vi "Galvo-Control-V3.vi"() -> ()   [LabVIEW 2024]
uses:
  <vilib>/DAQmx/write.llb/DAQmx Write (Analog 2D DBL NChan NSamp).vi
  <vilib>/DAQmx/write.llb/DAQmx Write (Analog 1D DBL NChan 1Samp).vi
  <vilib>/DAQmx/create/channels.llb/DAQmx Create Channel (AO-Voltage-Basic).vi
  <vilib>/DAQmx/miscellaneous.llb/DAQmx Fill In Error Info.vi
  <vilib>/measure/NI_MABase.lvlib
panel:
  out "element":dbl
  out "size(s)":i32
  out "Random Data (Feedback Node) 3":dbl[](graph)
  out "Random Data (Feedback Node) 2":dbl[](graph)
  out "Random Data (Feedback Node)":dbl[](graph)
  out "Y MIN":dbl
  out "Y MAX":dbl
  out "X MIN":dbl
  out "X MAX":dbl
  out "Waveform Chart":waveform(dbl)(graph)
  out "Waveform Chart 2":waveform(dbl)(graph)
  in  "offset X":dbl format="%0.2p"
  in  "amplitude X":dbl=1.0 format="%0.2p"
  in  "phase":dbl format="%.2p"
  in  "amplitude Y":dbl=1.0 format="%0.2p"
  in  "phase 2":dbl format="%.2p"
  in  "offset Y":dbl format="%0.2p"
  in  "COMMENCE SCAN":bool
  in  "Y desired voltage step(V/100)":dbl=1.0 format="%#_13g"
  in  "X desired voltage step(V/100)":dbl=1.0 format="%#_13g"
  out "Virtual Y position":dbl(graph)
  out "virtual X position":dbl(graph)
  out "Y position":dbl
  out "X position.":dbl
  # "This VI is intended for the user to first define a\nrectangular region to scan, and then to commence\nthe scan at some desired resolution.\n\nthe resolution is defined using the voltage step controls\n\nthe amplitude and offset controls define the scan region"
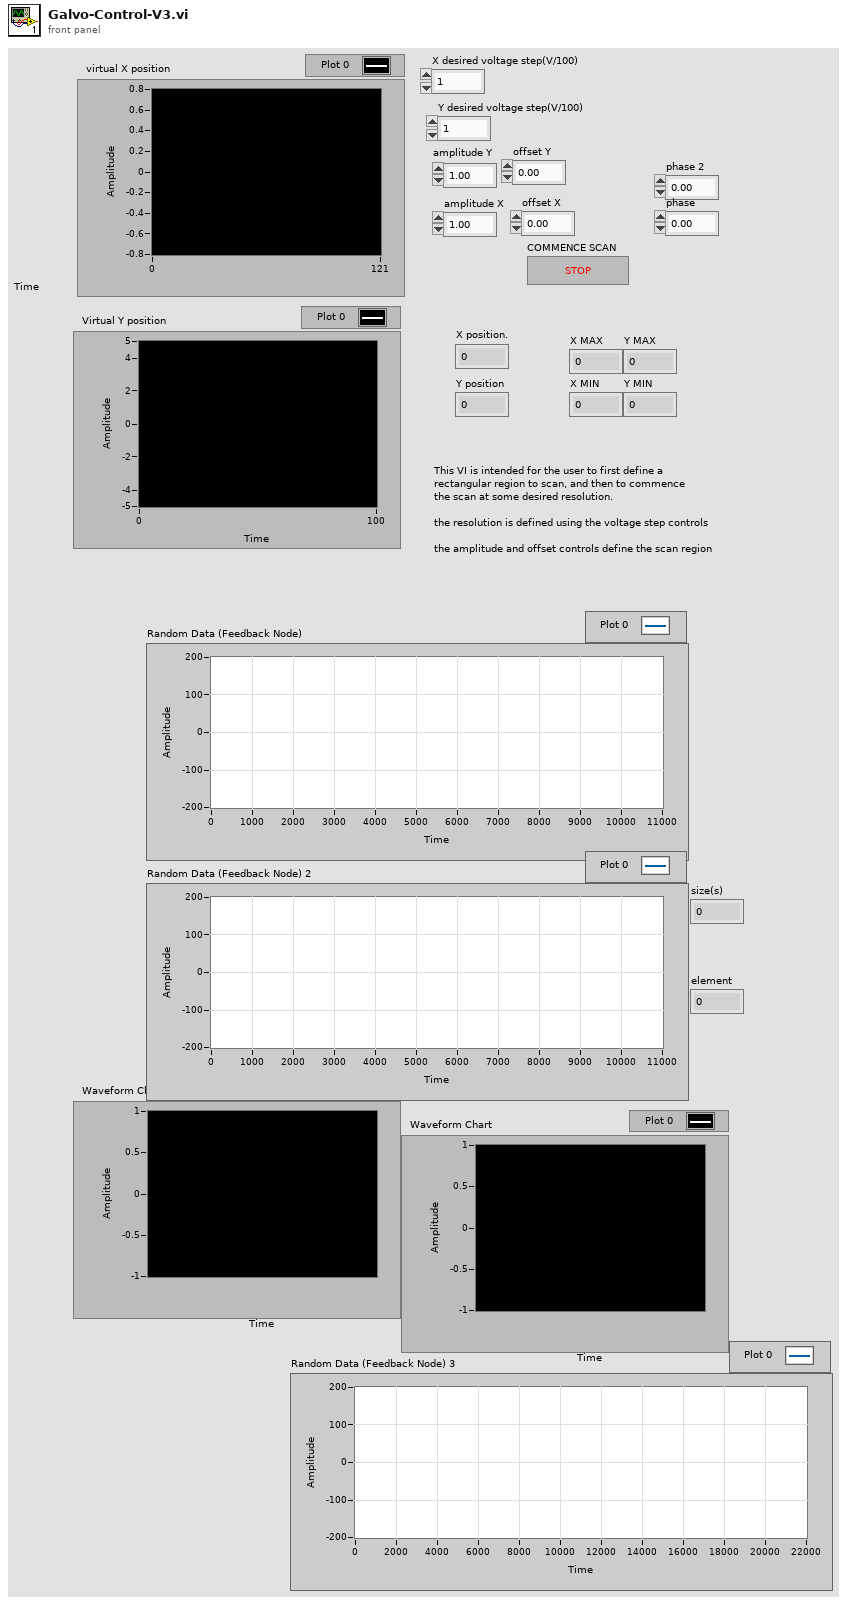
[diagram p1: front panel]
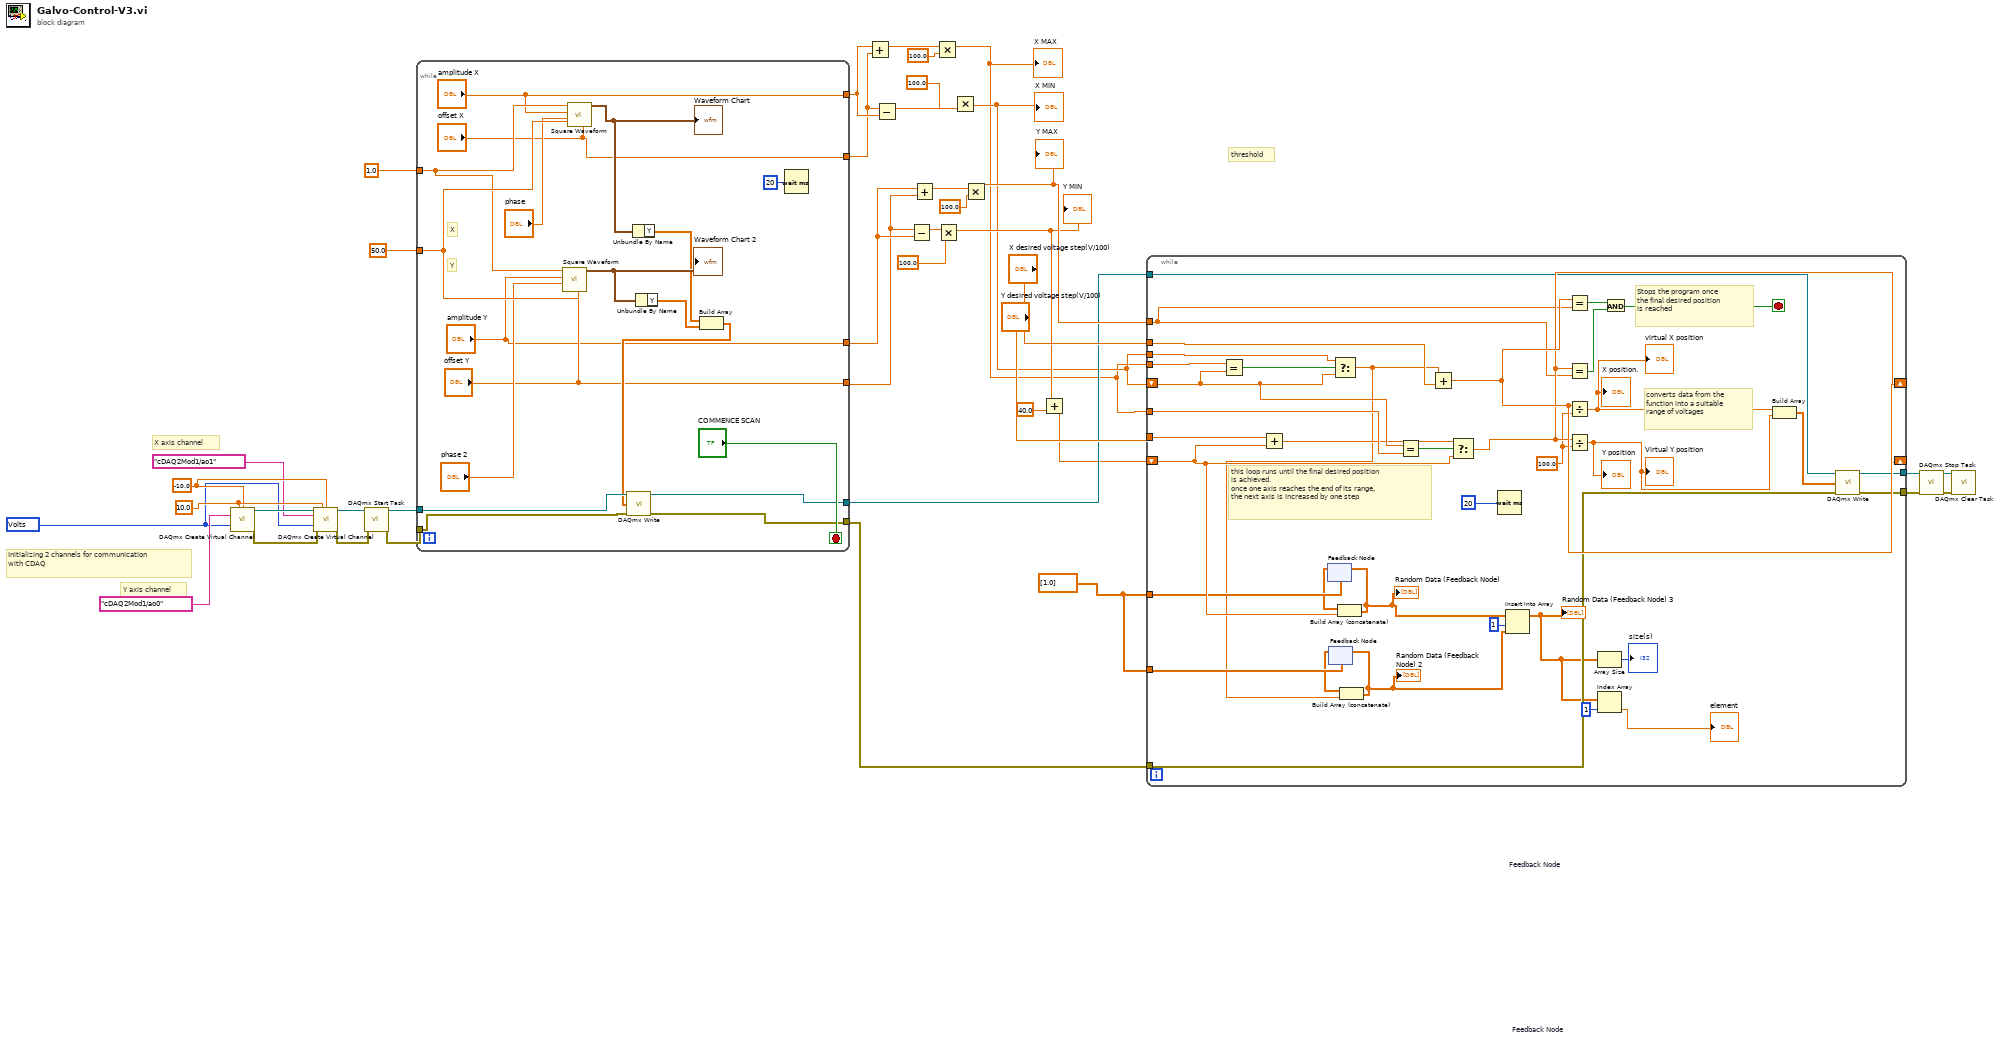
[diagram p0: block diagram]
diagram:
  w1 = dbl[] [1.0]
  w26 = 10348 items=["Volts"=10348, "From Custom Scale"=10065] ("units")
  w30 = 10.0 ("maximum value")
  w29 = -10.0 ("minimum value")
  # "Initializing 2 channels for communication\nwith CDAQ"
  # "X axis channel"
  # "Y axis channel"
  # "threshold"
  n1 = call-poly <vilib>:"DAQmx Create Virtual Channel.vi"("maximum value"=w30, "minimum value"=w29, "physical channels"=tag "cDAQ2Mod1/ao0", "units"=w26) -> ("task out"=w32:refnum<k21>, "error out"=w31:errorcluster)  [unwired: 10 in]
  n2 = call-poly <vilib>:"DAQmx Create Virtual Channel.vi"("task in"=w32, "maximum value"=w30, "minimum value"=w29, "physical channels"=tag "cDAQ2Mod1/ao1", "units"=w26, "error in"=w31) -> ("task out"=w25:refnum<k21>, "error out"=w24:errorcluster)  [unwired: 8 in]
  n3 = call <vilib>:"DAQmx Start Task.vi"("task/channels in"=w25, "error in"=w24) -> ("task out"=w23:refnum<k21>, "error out"=w22:errorcluster)  [unwired: 12 in]
  n4 = while {
    tunnel: 50.0 ("duty cycle (%)") -> [w59]
    tunnel: 1.0 ("frequency") -> [w58]
    tunnel: w23 -> [w53]
    tunnel: w22 -> [w52]
    tunnel: [w46] -> w18
    tunnel: [w45] -> w17
    tunnel: ["offset X"] -> w6
    tunnel: ["amplitude X"] -> w11
    tunnel: ["offset Y"] -> w4
    tunnel: ["amplitude Y"] -> w9
    stop <- "COMMENCE SCAN" stop-if-true
    # "Y"
    # "X"
    n5 = call <vilib>:"Square Waveform.vi"("duty cycle (%)"=w59, "offset"="offset Y", "phase"="phase 2", "amplitude"="amplitude Y", "frequency"=w58) -> ("signal out"=w51:waveform(dbl))  [unwired: 5 in, 1 out]
    "Waveform Chart 2" <- w51
    n6 = call <vilib>:"Square Waveform.vi"("duty cycle (%)"=w59, "offset"="offset X", "phase"="phase", "amplitude"="amplitude X", "frequency"=w58) -> ("signal out"=w50:waveform(dbl))  [unwired: 5 in, 1 out]
    "Waveform Chart" <- w50
    n7 = Unbundle By Name(w50) -> ("Y"=w49:dbl[])
    n8 = Unbundle By Name(w51) -> ("Y"=w48:dbl[])
    n9 = Build Array(w49, w48) -> (w47:dbl[][])
    n10 = call-poly <vilib>:"DAQmx Write.vi"("task/channels in"=w53, "data"=w47, "error in"=w52) -> ("task out"=w46:refnum<k21>, "error out"=w45:errorcluster)  [unwired: 10 in, 1 out]
    n11 = Wait (ms)(milliseconds to wait=u32 20) -> ()  [unwired: 1 out]
  }
  n12 = Add(x=w11, y=w6) -> (x+y=w7:dbl)
  n13 = Subtract(x=w6, y=w11) -> (x-y=w12:dbl)
  n14 = Subtract(x=w4, y=w9) -> (x-y=w10:dbl)
  n15 = Add(x=w9, y=w4) -> (x+y=w5:dbl)
  n16 = Multiply(x=w7, y=100.0) -> (x*y=w8:dbl)
  "X MAX" <- w8
  n17 = Multiply(x=w10, y=100.0) -> (x*y=w16:dbl)
  "Y MIN" <- w16
  n18 = Multiply(x=w12, y=100.0) -> (x*y=w14:dbl)
  "X MIN" <- w14
  n19 = Multiply(x=w5, y=100.0) -> (x*y=w20:dbl)
  "Y MAX" <- w20
  n20 = Add(x=w16, y=40.0) -> (x+y=w2:dbl)
  n21 = while {
    shift-right: [w91] -> _
    shift-left: w14 -> [w96]
    shift-right: [w90] -> _
    shift-left: w2 -> [w95]
    tunnel: [w85] -> w40
    tunnel: [w84] -> w39
    tunnel: w18 -> [w83]
    tunnel: w17 -> [w82]
    tunnel: "Y desired voltage step(V/100)" -> [w81]
    tunnel: "X desired voltage step(V/100)" -> [w80]
    tunnel: w8 -> [w79]
    tunnel: w8 -> [w78]
    tunnel: w20 -> [w77]
    tunnel: w14 -> [w76]
    tunnel: w1 -> [w75]
    tunnel: w1 -> [w74]
    stop <- w92 stop-if-true
    w89 = 100.0 ("x")
    # "this loop runs until the final desired position\nis achieved.\nonce one axis reaches the end of its range,\nthe next axis is increased by one step"
    # "converts data from the\nfunction into a suitable \nrange of voltages"
    # "Stops the program once\nthe final desired position \nis reached"
    n22 = Equal?(x=w79, y=w96) -> (x = y?=w73:bool)
    n23 = Add(x=w81, y=w95) -> (x+y=w70:dbl)
    n24 = feedback #1 "Feedback Node"(w75) -> (w69:dbl[])
    n25 = feedback #2 "Feedback Node"(w74) -> (w68:dbl[])
    n26 = Select(t=w76, s=w73, f=w96) -> (s? t:f=w67:dbl)
    n27 = Build Array (concatenate)(w69, w95) -> (w66:dbl[])
    "Random Data (Feedback Node)" <- w66
    n28 = feedback-in #1(w66) -> ()
    n29 = Build Array (concatenate)(w68, w67) -> (w65:dbl[])
    "Random Data (Feedback Node) 2" <- w65
    n30 = feedback-in #2(w65) -> ()
    n31 = Equal?(x=w96, y=w78) -> (x = y?=w72:bool)
    n32 = Add(x=w67, y=w80) -> (x+y=w91:dbl)
    n33 = Select(t=w70, s=w72, f=w95) -> (s? t:f=w90:dbl)
    n34 = Wait (ms)(milliseconds to wait=u32 20) -> ()  [unwired: 1 out]
    n35 = Insert Into Array(array=w66, index=1, new element=w65) -> (w62:dbl[])
    "Random Data (Feedback Node) 3" <- w62
    n36 = Equal?(x=w91, y=w77) -> (x = y?=w94:bool)
    n37 = Equal?(x=w90, y=w77) -> (x = y?=w93:bool)
    n38 = Divide(x=w91, y=w89) -> (x/y=w87:dbl)
    "X position." <- w87
    "virtual X position" <- w87
    n39 = Divide(x=w90, y=w89) -> (x/y=w88:dbl)
    "Y position" <- w88
    "Virtual Y position" <- w88
    n40 = Array Size(array=w62) -> (size(s)=→"size(s)":i32)
    n41 = Index Array(array=w62, index=1) -> (element=→"element":dbl)
    n42 = And(x=w94, y=w93) -> (x .and. y?=w92:bool)
    n43 = Build Array(w87, w88) -> (w86:dbl[])
    n44 = call-poly <vilib>:"DAQmx Write.vi"("task/channels in"=w83, "data"=w86, "error in"=w82) -> ("task out"=w85:refnum<k21>, "error out"=w84:errorcluster)  [unwired: 10 in, 1 out]
  }
  n45 = call <vilib>:"DAQmx Stop Task.vi"("task/channels in"=w40, "error in"=w39) -> ("task out"=w38:refnum<k21>, "error out"=w37:errorcluster)  [unwired: 12 in]
  n46 = call <vilib>:"DAQmx Clear Task.vi"("task in"=w38, "error in"=w37) -> ()  [unwired: 13 in, 1 out]
